vi "Matrix_LltDecompose.vi"(10 "LowerTriangle":bool, 11 "input matrix":T1) -> (0 "Error":bool, 3 "output Cholesky Decomp":T1)   [LabVIEW 2019, in "Trajectory_Library.lvlib"]
doc: "Decompose \"this\" matrix using Cholesky Decomposition. If the \"this\" matrix is zeros, it will return the zero matrix.\n \nInputs:\n - input matrix -- The input matrix\n - lowerTriangular -- Whether or not we want to decompose to the lower triangular Cholesky matrix.\n\nOutputs:\n - output Cholesky Decomp -- The decomposed matrix.\n - error -- If TRUE, an error occured. For example if the matrix could not be decomposed(ie. is not positive semidefinite."
uses:
  Trajectory_Library.lvlib
  <vilib>/Analysis/NI_AALPro.lvlib
  <vilib>/Analysis/7linalg.llb/Real Cholesky Factorization.vi
  <vilib>/Analysis/Matrix/Datatypes/RealMatrix.ctl
  <vilib>/Analysis/Matrix/NI_Matrix.lvlib
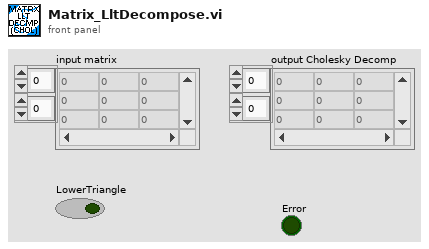
[diagram p1: front panel]
types:
  T1 = typedef "NI_Matrix.lvlib/RealMatrix.ctl" = dbl[][]
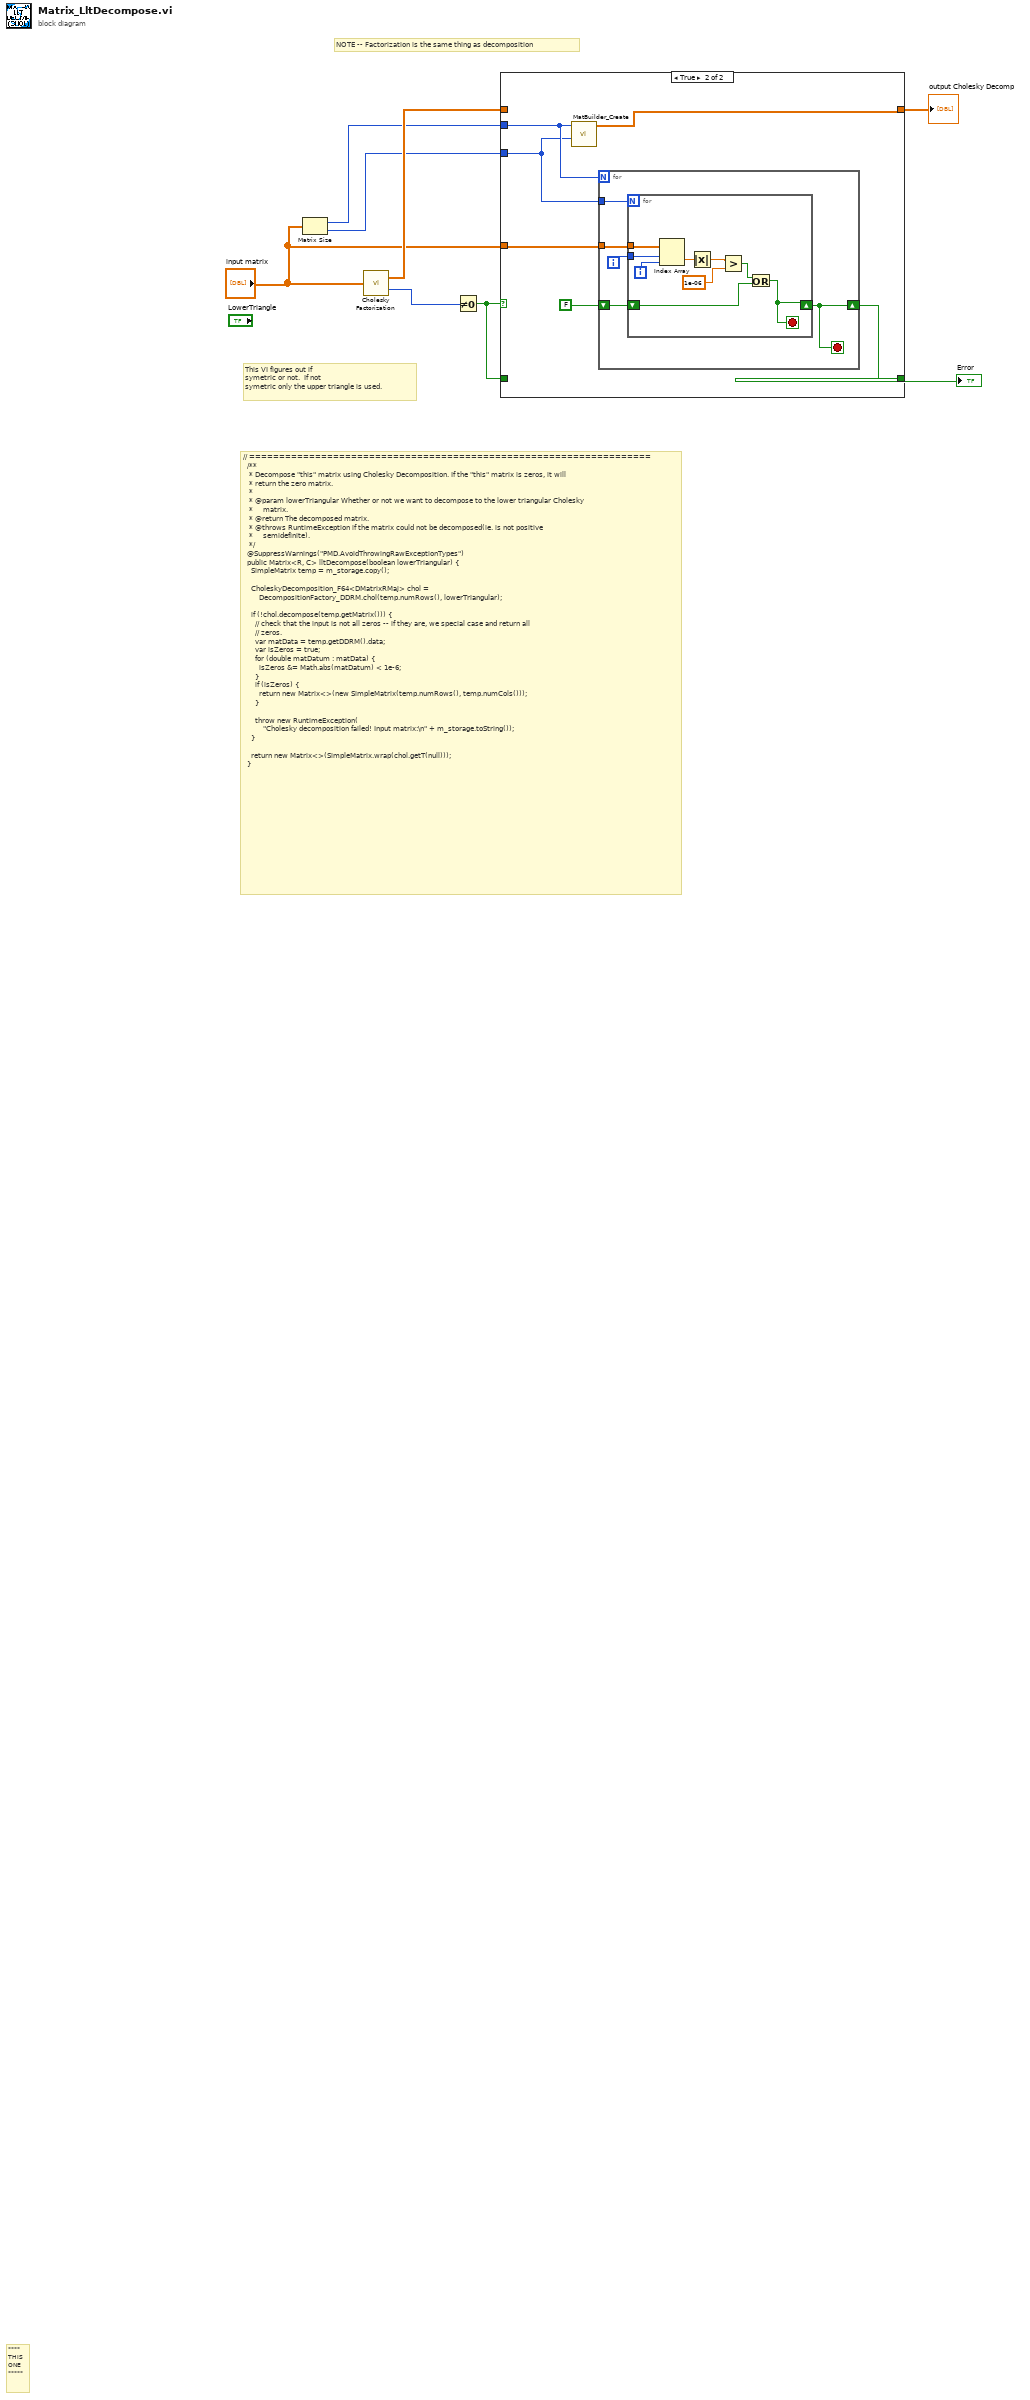
[diagram p0: block diagram]
diagram:
  # "This VI figures out if\nsymetric or not.  If not \nsymetric only the upper triangle is used."
  # "NOTE -- Factorization is the same thing as decomposition"
  # "// ===================================================================\n  /**\n   * Decompose \"this\" matrix using Cholesky Decomposition. If the \"this\" matrix is zeros, it will\n   * return the zero matrix.\n   *\n   * @param lowerTriangular Whether or not we want to decompose to the lower triangular Cholesky\n   *     matrix.\n   * @return The decomposed matrix.\n   * @throws RuntimeException if the matrix could not be decomposed(ie. is not positive\n   *     semidefinite).\n   */\n  @SuppressWarnings(\"PMD.AvoidThrowingRawExceptionTypes\")\n  public Matrix<R, C> lltDecompose(boolean lowerTriangular) {\n    SimpleMatrix temp = m_storage.copy();\n\n    CholeskyDecomposition_F64<DMatrixRMaj> chol =\n        DecompositionFactory_DDRM.chol(temp.numRows(), lowerTriangular);\n\n    if (!chol.decompose(temp.getMatrix())) {\n      // check that the input is not all zeros -- if they are, we special case and return all\n      // zeros.\n      var matData = temp.getDDRM().data;\n      var isZeros = true;\n      for (double matDatum : matData) {\n        isZeros &= Math.abs(matDatum) < 1e-6;\n      }\n      if (isZeros) {\n        return new Matrix<>(new SimpleMatrix(temp.numRows(), temp.numCols()));\n      }\n\n      throw new RuntimeException(\n          \"Cholesky decomposition failed! Input matrix:\\n\" + m_storage.toString());\n    }\n\n    return new Matrix<>(SimpleMatrix.wrap(chol.getT(null)));\n  }"
  # "****\nTHIS\nONE\n*****"
  n1 = Matrix Size(0:"input matrix") -> (1:w3:i32, 2:w2:i32)
  n2 = call-poly <vilib>:"Cholesky Factorization.vi"("A"="input matrix") -> ("Cholesky"=w7:T1, "error"=w8:i32)
  n3 = Not Equal To 0?(x=w8) -> (x != 0?=w5:bool)
  n4 = case shown="True" w5 {
    tunnel: [w10 w16] -> w6
    tunnel: w7 -> [w10 _]
    tunnel: w5 -> [w9 _]
    tunnel: [w9 w11] -> w4
    tunnel: w3 -> [_ w15]
    tunnel: w2 -> [_ w14]
    tunnel: "input matrix" -> [_ w13]
    frame False {
    }
    frame True {
      n5 = call "MatBuilder_Create.vi"("Columns"=w14, "Rows"=w15) -> ("output matrix"=w16:T1)  [unwired: 9 in]
      n6 = for {
        N: w15 -> [_]
        tunnel: w14 -> [w21]
        tunnel: w13 -> [w19]
        shift-right: [w17] -> w11
        shift-left: FALSE -> [w18]
        i -> [w20]
        stop <- w17 stop-if-true
        n7 = for {
          N: w21 -> [_]
          tunnel: w20 -> [w30]
          tunnel: w19 -> [w28]
          shift-right: [w22] -> w17
          shift-left: w18 -> [w23]
          i -> [w29]
          stop <- w22 stop-if-true
          n8 = Index Array(array=w28, index (row)=w30, index (col)=w29) -> (element=w27:dbl)
          n9 = Absolute Value(x=w27) -> (abs(x)=w26:dbl)
          n10 = Greater?(x=w26, y=1e-06) -> (0:w24:bool)
          n11 = Or(x=w24, y=w23) -> (x .or. y?=w22:bool)
        }
      }
    }
  }
  "output Cholesky Decomp" <- w6
  "Error" <- w4
